vi "Initialize.vi"(8 "error in":errorcluster, 11 "Plugin in":refnum<class "Nominal-Streamer.lvclass">) -> (0 "error out":errorcluster, 3 "Plugin out":refnum<class "Nominal-Streamer.lvclass">)   [LabVIEW 2020, in "Nominal-Streamer.lvlib" / "Nominal-Streamer.lvclass"]
doc: "Initializes the plugin, creating several parameters."
uses:
  Nominal-Streamer.lvclass
  <vilib>/FlexLogger/SDK/PluginSDK.lvlibp/PEFClasses/SDK/Plugin/Plugin.lvclass
  <vilib>/FlexLogger/SDK/PluginSDK.lvlibp/PEFClasses/SDK/System Interface/Resampling Mode.ctl
  <vilib>/FlexLogger/SDK/PluginSDK.lvlibp/PEFClasses/SDK/System Interface/System Interface.lvclass
  <vilib>/FlexLogger/SDK/PluginSDK.lvlibp/PEFClasses/SDK/Processing Element/Timing Method.ctl
  <vilib>/FlexLogger/SDK/PluginSDK.lvlibp/PEFClasses/SDK/Processing Element/Processing Element.lvclass
  <vilib>/FlexLogger/SDK/PluginSDK.lvlibp/PEFClasses/SDK/Processing Element/Timing Parameters.ctl
  <vilib>/FlexLogger/SDK/PluginSDK.lvlibp/PEFClasses/SDK/Plugin/ParameterAccess/Write String.vi
  <vilib>/FlexLogger/SDK/PluginSDK.lvlibp/PEFClasses/SDK/Plugin/ParameterAccess/Write N Channel.vi
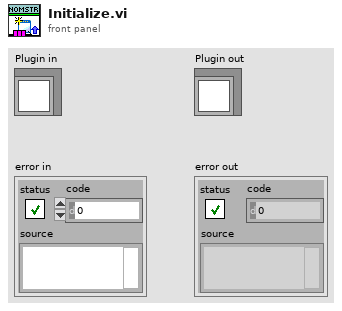
[diagram p1: front panel]
types:
  T1 = typedef "PluginSDK.lvlibp/Processing Element.lvclass/Timing Parameters.ctl" = cluster{"Timing Method":T2, "Timing Period (ms)":i32}
  T2 = typedef "PluginSDK.lvlibp/Processing Element.lvclass/Timing Method.ctl" = enum16{"Periodic", "Immediate", "On Data Ready", "Triggered"}
  T3 = typedef "PluginSDK.lvlibp/System Interface.lvclass/Resampling Mode.ctl" = enum16{"No Resampling", "Custom Rate", "Maximum Rate", "Minimum Rate"}
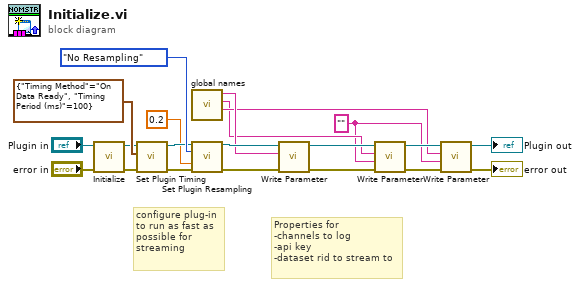
[diagram p0: block diagram]
diagram:
  w8 = "" ("Value")
  # "configure plug-in to run as fast as possible for streaming"
  # "Properties for\n-channels to log\n-api key\n-dataset rid to stream to"
  n1 = call-parent "Initialize.vi"("error in (no error)"="error in", "Plugin in"="Plugin in") -> ("error out"=w6:errorcluster, "Plugin out"=w3:refnum<class "Nominal-Streamer.lvclass">)  [unwired: 8 in]
  n2 = call <vilib>:"Set Plugin Timing.vi"("error in (no error)"=w6, "Timing Parameters"=T1 {"Timing Method"=enum."On Data Ready", "Timing Period (ms)"=100}, "Plugin in"=w3) -> ("error out"=w16:errorcluster, "Plugin out"=w15:refnum<class "Nominal-Streamer.lvclass">)  [unwired: 7 in]
  n3 = call "global names.vi"() -> ("dataset RID"=w10:string, "API Key"=w9:string, "logged channels name"=w17:string)  [unwired: 9 in]
  n4 = call <vilib>:"Set Plugin Resampling.vi"("Plugin in"=w15, "Resampling Mode"=Resampling_Mode."No Resampling", "Block Size (s)"=0.2, "error in (no error)"=w16) -> ("Plugin out"=w21:refnum<class "Nominal-Streamer.lvclass">, "error out"=w20:errorcluster)  [unwired: 10 in]
  n5 = call-poly <vilib>:"Write Parameter.vi"("error in (no error)"=w20, "Name (Unique Channel Identifier)"=w17, "Plugin in"=w21) -> ("error out"=w19:errorcluster, "Plugin out"=w12:refnum<class "Nominal-Streamer.lvclass">)  [unwired: 7 in]
  n6 = call-poly <vilib>:"Write Parameter.vi"("error in (no error)"=w19, "Value"=w8, "Name"=w9, "Plugin in"=w12) -> ("error out"=w13:errorcluster, "Plugin out"=w11:refnum<class "Nominal-Streamer.lvclass">)  [unwired: 6 in]
  n7 = call-poly <vilib>:"Write Parameter.vi"("error in (no error)"=w13, "Value"=w8, "Name"=w10, "Plugin in"=w11) -> ("error out"=→"error out":errorcluster, "Plugin out"=→"Plugin out":refnum<class "Nominal-Streamer.lvclass">)  [unwired: 6 in]
